vi "Tag Engine Test 1.vi"() -> ()   [LabVIEW 2020]
doc: "_Test_"
uses:
  Tag/Tag.lvclass/Tag.ctl
  a32eeae9-b076-4228-86a7-a13287abedbe.vi
  20c6578c-4bd2-4559-8eb7-19bb61ff37ef.vi
  d7e5d0a7-9399-4335-9200-169007c2c370.vi
  e3e97c5d-b2e9-4921-842e-d8e3f4c8e528.vi
  5595b3a8-0848-405d-a2a8-398ae7258ff6.vi
  931b2265-17ad-46e4-91be-eaf1127382fd.vi
  Tag/Construct.vi
  API/Get Tag Value_ByRef.vi
  Tag/Read Value.vi
  Tag/Read Timestamp.vi
  Core/Get Delimiter.vi
  <vilib>/Utility/error.llb/Error Cluster From Error Code.vi
  Tag/Set Properties from Initial.vi
  Core/Add Tag.vi
  <vilib>/Utility/Data Type/Get Type Information.vi
  <vilib>/JDP Science/JSONtext/Variant to JSON Text.vi
  Tag/Tag.lvclass
  Tag Engine.lvlib
panel:
  in  "Value2":dbl[][][](array[numeric])=[[[1.0, 2.0], [3.0, 4.0]], [[1.0, 1.0], [1.0, 1.0]]]
  out "Value1 (Strict)":cluster{"test1":i32, "test2":dbl}
  in  "Value1":cluster{"test1":i32, "test2":dbl}={"test1"=1, "test2"=2.0}
  out "Value2 (Variant)":variant
  out "Value2 (As String)":string
  out "Value2 (Strict)":dbl[][][](array[numeric])
  out "Value1 (Variant)":variant
  out "Value1 (As String)":string
  out "error out":errorcluster
  out "error out 2":errorcluster
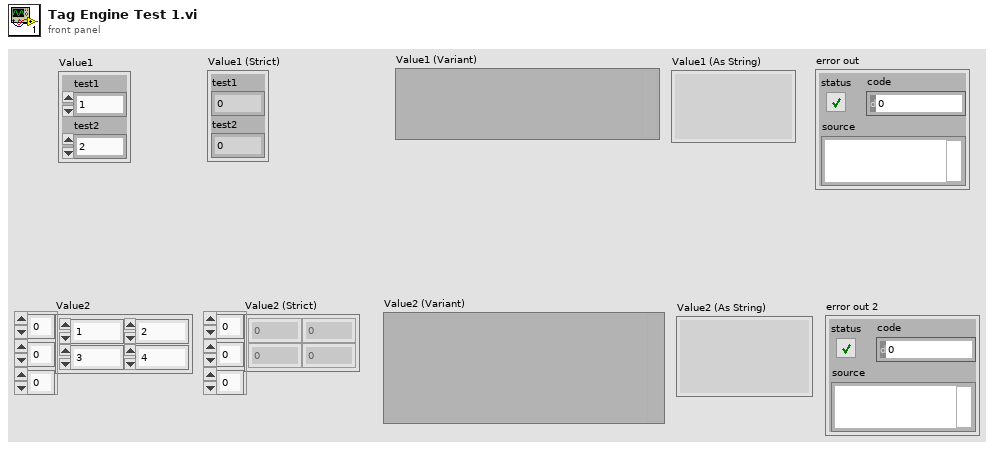
[diagram p1: front panel]
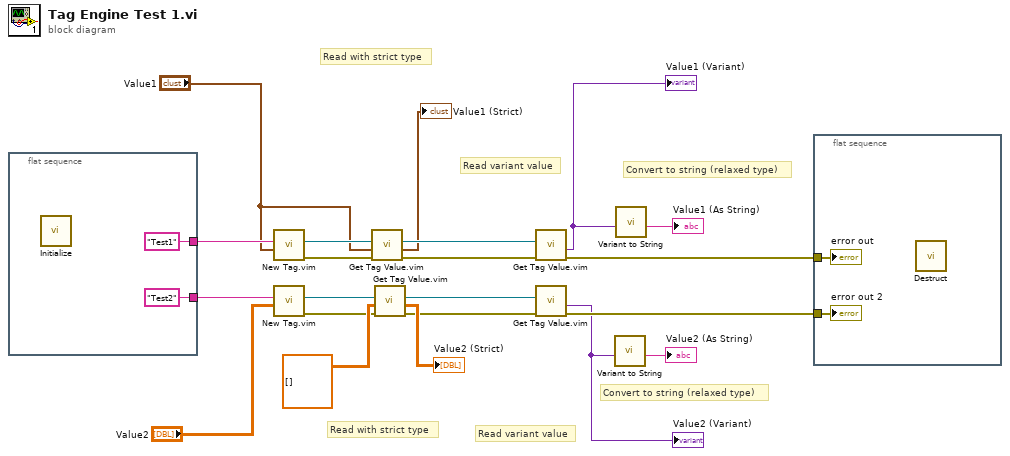
[diagram p0: block diagram]
diagram:
  # "Read variant value"
  # "Read with strict type"
  # "Convert to string (relaxed type)"
  # "Read variant value"
  # "Convert to string (relaxed type)"
  # "Read with strict type"
  n1 = flat-sequence {
    tunnel: ["Test1" ("Name")] -> w21
    tunnel: ["Test2" ("Name")] -> w20
    frame #0 {
      n2 = call "Initialize.vi"() -> ()  [unwired: 11 in, 1 out]
    }
  }
  n3 = call "New Tag.vim"("Initial Value"="Value1", "Tag Name"=w21) -> ("error out"=w18:errorcluster, "Tag Ref out"=w19:refnum<data-value>)  [unwired: 8 in]
  n4 = call "New Tag.vim"("Initial Value"="Value2", "Tag Name"=w20) -> ("error out"=w11:errorcluster, "Tag Ref out"=w13:refnum<data-value>)  [unwired: 8 in]
  n5 = call "Get Tag Value.vim"("error in (no error)"=w18, "Default (Void)"="Value1", "Tag Name(s)/Ref(s)"=w19) -> ("error out"=w16:errorcluster, "Value(s)"=→"Value1 (Strict)":cluster{"test1":i32, "test2":dbl}, "Tag Ref(s) out"=w17:refnum<data-value>)  [unwired: 5 in, 1 out]
  n6 = call "Get Tag Value.vim"("error in (no error)"=w11, "Default (Void)"=dbl[][][] [], "Tag Name(s)/Ref(s)"=w13) -> ("error out"=w10:errorcluster, "Value(s)"=→"Value2 (Strict)":dbl[][][], "Tag Ref(s) out"=w9:refnum<data-value>)  [unwired: 5 in, 1 out]
  n7 = call "Get Tag Value.vim"("error in (no error)"=w16, "Tag Name(s)/Ref(s)"=w17) -> ("error out"=w1:errorcluster, "Value(s)"=w5:variant)  [unwired: 6 in, 2 out]
  "Value1 (Variant)" <- w5
  n8 = call "Get Tag Value.vim"("error in (no error)"=w10, "Tag Name(s)/Ref(s)"=w9) -> ("error out"=w6:errorcluster, "Value(s)"=w4:variant)  [unwired: 6 in, 2 out]
  "Value2 (Variant)" <- w4
  n9 = call "Variant to String.vi"("Variant Value"=w4) -> ("String Value"=→"Value2 (As String)":string)  [unwired: 9 in, 1 out]
  n10 = call "Variant to String.vi"("Variant Value"=w5) -> ("String Value"=→"Value1 (As String)":string)  [unwired: 9 in, 1 out]
  n11 = flat-sequence {
    tunnel: w6 -> [w25]
    tunnel: w1 -> [w24]
    frame #0 {
      n12 = call "Destruct.vi"() -> ()  [unwired: 11 in, 1 out]
      "error out 2" <- w25
      "error out" <- w24
    }
  }
